vi "Set Display Format and units Method.vi"(0 "Display State In":T1, 1 "Units":string, 5 "digits":i32, 7 "sf(F) or dp ?":bool, 9 "Container State":T2, 11 "error in (no error)":errorcluster) -> (4 "Display State Out":T1, 15 "error out":errorcluster)   [LabVIEW 2012, in "Vector Function Generator.xctl"]
doc: "Method to store display format preferences for the waveform controls into our volatile state"
uses:
  Vector Function Generator.xctl
  <vilib>/_xctls/Container State.ctl
  Vector State.ctl
  <vilib>/_xctls/XControlSupport.lvlib
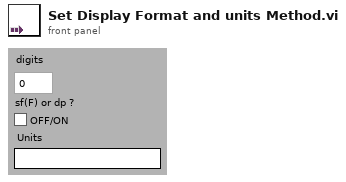
[diagram p1: front panel]
types:
  T1 = typedef "Vector Function Generator.xctl/Vector State.ctl" = cluster{"Current Position":i32, "Show Current Position":bool, "Mode (F=Polar)":bool, "digits":i32, "sf(F) or dp ?":bool, "Units":string}
  T2 = typedef "XControlSupport.lvlib/Container State.ctl" = cluster{"Indicator?":bool, "Run Mode?":bool, " Refnum":refnum<vi>}
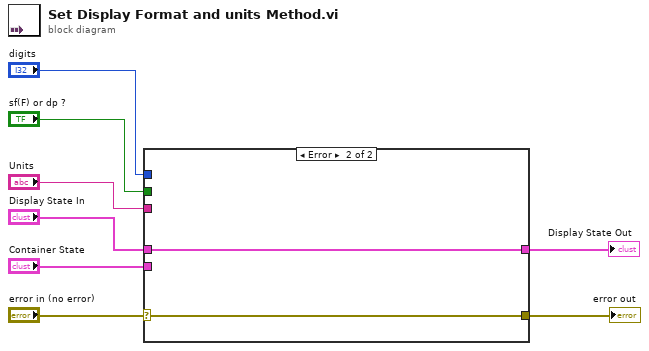
[diagram p0: block diagram]
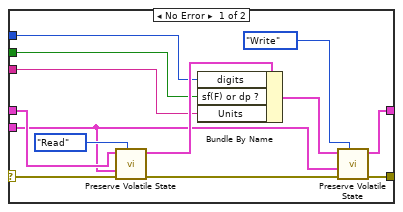
[diagram p2: hidden frame]
diagram:
  n1 = case shown="Error" "error in (no error)" {
    selector: "error in (no error)" -> [w19 w22]
    tunnel: "Display State In" -> [w21 w23]
    tunnel: "Container State" -> [w16 _]
    tunnel: [w14 w22] -> w5
    tunnel: "Units" -> [w13 _]
    tunnel: "sf(F) or dp ?" -> [w12 _]
    tunnel: "digits" -> [w11 _]
    tunnel: [w10 w23] -> w1
    frame No Error {
      n2 = call "Preserve Volatile State.vi"("Operation In"=enum16{"Read", "Write", "Update From Data"}."Read" ("Operation"), "Error In (no Error) In"=w19, "Container State In"=w16, "Waveform State In"=w21) -> ("Error Out"=w15:errorcluster, "Waveform State Out"=w18:T1)  [unwired: 1 in, 5 out]
      n3 = Bundle By Name(cluster=w18, "digits"=w11, "sf(F) or dp ?"=w12, "Units"=w13) -> (w17:T1)
      n4 = call "Preserve Volatile State.vi"("Operation In"=enum16{"Read", "Write", "Update From Data"}."Write" ("Operation"), "Error In (no Error) In"=w15, "Container State In"=w16, "Waveform State In"=w17) -> ("Error Out"=w14:errorcluster, "Waveform State Out"=w10:T1)  [unwired: 1 in, 5 out]
    }
    frame Error {
    }
  }
  "Display State Out" <- w1
  "error out" <- w5
